vi "Main.vi"(11 "Module Admin":refnum<class "Delacor_lib_QMH_Cloneable Module Admin.lvclass">) -> ()   [LabVIEW 2020, in "reporting-device.lvlib"]
doc: "This template is based off of the Queued Message Handler design pattern and the Queued Message Handler project template that ships with LabVIEW.\n\nThe main difference is that the queue is private to this module and communication between modules is performed via Broadcast and Request events.\n\nRequest events are wrapped in public API methods and are handled in the Event Handling Loop (EHL) of this VI. Any module can register for Broadcast events sent by this module. The EHL generates messages based on user interface actions.\n\nThe Message Handling Loop (MHL) processes messages generated by the EHL, or by other messages. The messages are string values, so new messages can be added easily to the Message Cases case structure in the MHL. Each message cluster can also provide an optional value for Message Data, which is a variant that can be converted to whatever message-specific data is required.\n_____\nBased on DQMH Project Template 7.0.1.1316."
uses:
  reporting-device.lvlib
  <vilib>/Delacor/Delacor QMH/Libraries/Message Queue_class/Delacor_lib_QMH_Message Queue.lvclass
  <vilib>/Utility/miscctls.llb/LVPointTypeDef.ctl
  <vilib>/Delacor/Delacor QMH/Libraries/Message Queue_class/Delacor_lib_QMH_Enqueue Message (Single).vi
  Stop Argument--cluster.ctl
  <vilib>/Delacor/Delacor QMH/Libraries/Cloneable Module Admin_class/Delacor_lib_QMH_Cloneable Module Admin.lvclass
  connect (Reply Payload)--cluster.ctl
  connect Argument--cluster.ctl
  <userlib>/Zaphiro/GTools/Redis/Sources/Redis/Redis.lvclass
  <vilib>/Wovalab/Utilities/Helper Loop Periodic Timing/Helper Loop Periodic Timing.lvclass
  start-publishing (Reply Payload)--cluster.ctl
  start-publishing Argument--cluster.ctl
  <userlib>/Zaphiro/GTools/Time/time__ZGTools.lvlib
  <userlib>/Zaphiro/GTools/Time/public/convert lv time to unix-scalar__ZGTools.vi
  set-reporting-device (Reply Payload)--cluster.ctl
  set-reporting-device Argument--cluster.ctl
  <userlib>/Zaphiro/GTools/Time/public/convert unix time to lv-scalar__ZGTools.vi
panel:
  out "ttl":i32 format="%d s"
  out "values":dbl[](array[numeric])
  out "timestamp":timestamp format="%^<%x %.3X>T utc"
  out "latest-ts":u64
  out "info":T1
  out "status":string
  out "connected":bool
  out "error out":errorcluster
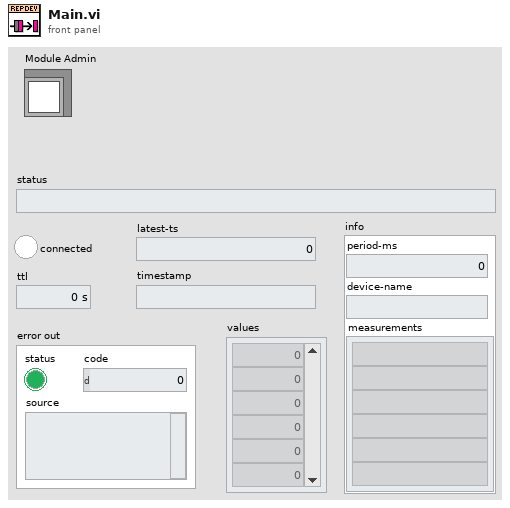
[diagram p1: front panel]
types:
  T1 = cluster{"period-ms":i32, "device-name":string, "measurements":string[]}
  T2 = typedef "reporting-device.lvlib/Request Events--cluster.ctl" = cluster{"Stop Module":refnum<user-event>, "Show Panel":refnum<user-event>, "Hide Panel":refnum<user-event>, "Show Diagram":refnum<user-event>, "Get Module Execution Status":refnum<user-event>, "connect":refnum<user-event>, "start-publishing":refnum<user-event>, "set-reporting-device":refnum<user-event>}
  T3 = typedef "reporting-device.lvlib/Module Data--cluster.ctl" = cluster{"clone-id":i32, "status":string, "dvr":cluster{"redis":refnum<data-value>}}
  T4 = enum32{"invalid lock state", "Not Locked", "Locked (No Password)", "Password-protected"}
  T5 = typedef "reporting-device.lvlib/Stop Argument--cluster.ctl" = cluster{"Module ID":i32, "Origin":string, "Exit via Stop Module Req?":bool, "Wait for Module to stop?":bool}
  T6 = typedef "reporting-device.lvlib/connect Argument--cluster.ctl" = cluster{"Module ID":i32, "flush":bool, "connection":cluster{"ip":string, "port":u16, "timeout":i32}, "Wait Notifier":refnum<notifier>, "wait for reply":bool}
  T7 = typedef "reporting-device.lvlib/start-publishing Argument--cluster.ctl" = cluster{"Module ID":i32, "Wait Notifier":refnum<notifier>, "wait for reply":bool}
  T8 = typedef "reporting-device.lvlib/set-reporting-device Argument--cluster.ctl" = cluster{"Module ID":i32, "measurement-list":string[], "period-ms":i32, "device-name":string, "ttl":i32, "Wait Notifier":refnum<notifier>, "wait for reply":bool}
  T9 = typedef "LVPointTypeDef.ctl" = cluster{"Horizontal":i16, "Vertical":i16}
  T10 = enum32{"Invalid", "Standard", "Closed", "Hidden", "Minimized", "Maximized"}
  T11 = typedef "reporting-device.lvlib/connect (Reply Payload)--cluster.ctl" = cluster{"Module ID":i32, "status":cluster{"reply-to-ping":bool, "pong":bool}, "error":errorcluster}
  T12 = typedef "reporting-device.lvlib/start-publishing (Reply Payload)--cluster.ctl" = cluster{"Module ID":i32, "ack":bool, "ts":u64, "error":errorcluster}
  T13 = typedef "reporting-device.lvlib/set-reporting-device (Reply Payload)--cluster.ctl" = cluster{"Module ID":i32, "ack":bool, "error":errorcluster}
  T14 = cluster{"output cluster":refnum<class "Redis.lvclass">}
  T15 = cluster{"period-ms":i32, "device-name":string, "measurement-list":string[]}
  T16 = cluster{u64, "device-name":string, "measurement-list":string[], "ttl":i32}
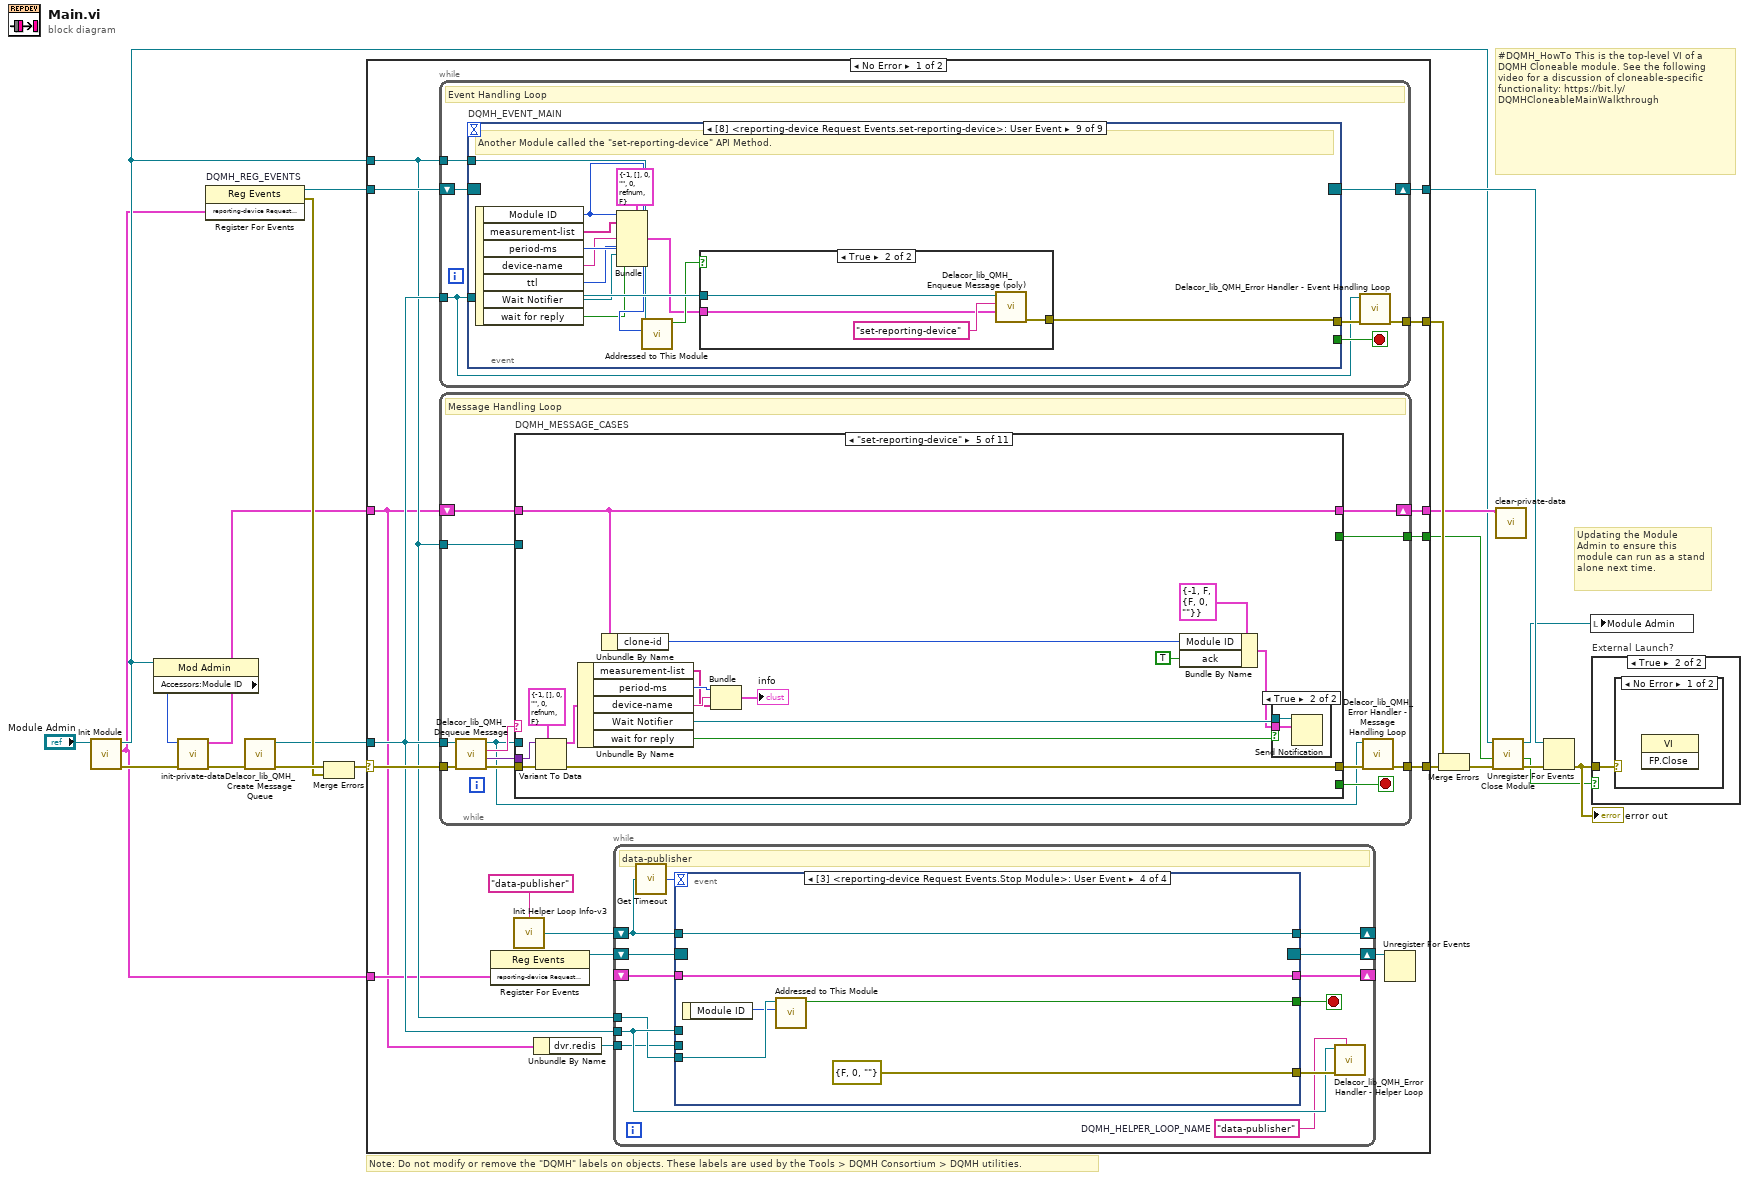
[diagram p0: block diagram]
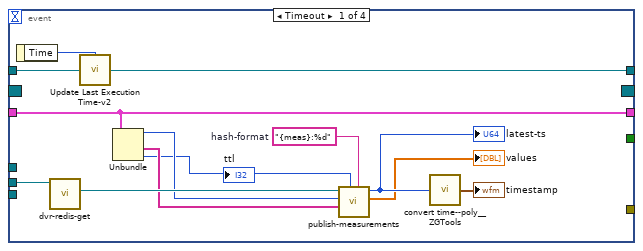
[diagram p2: hidden frame]
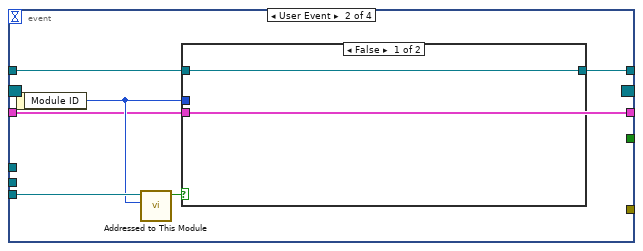
[diagram p3: hidden frame]
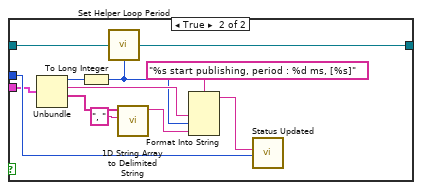
[diagram p4: hidden frame]
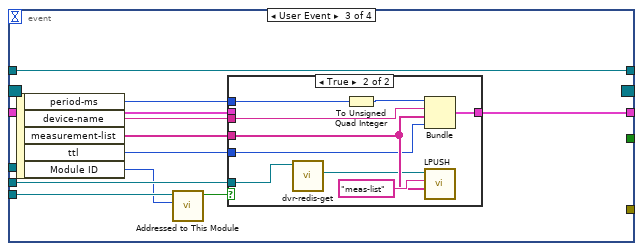
[diagram p5: hidden frame]
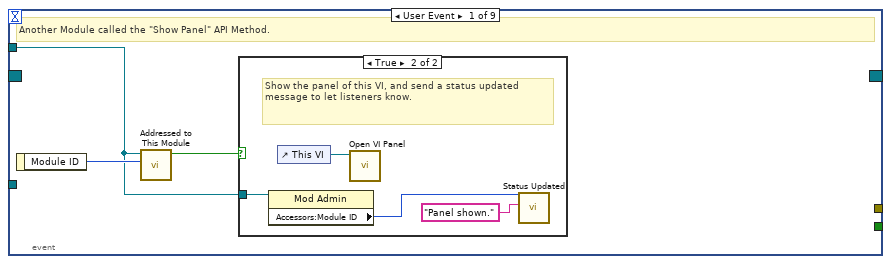
[diagram p7: hidden frame]
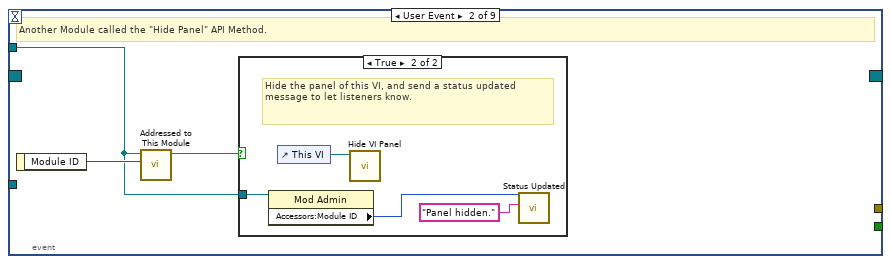
[diagram p9: hidden frame]
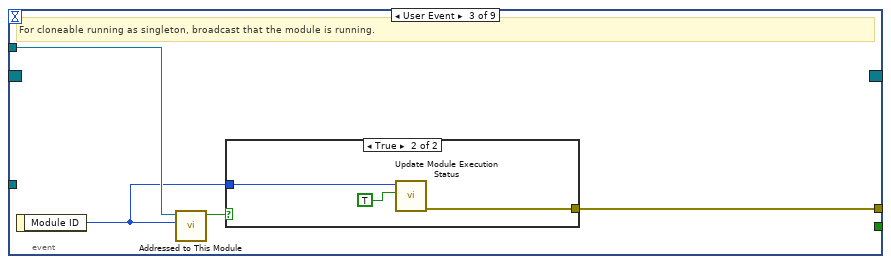
[diagram p11: hidden frame]
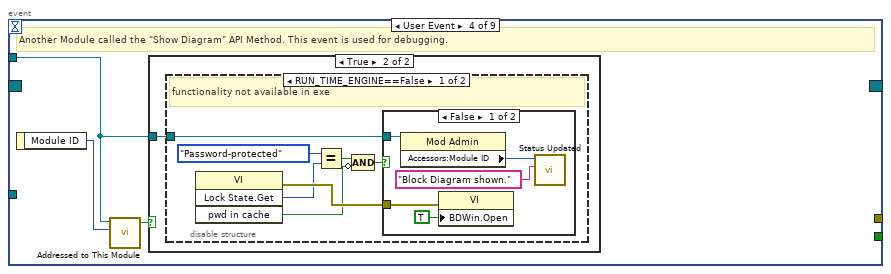
[diagram p13: hidden frame]
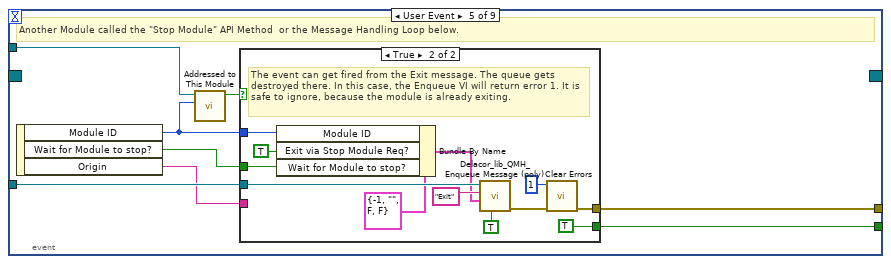
[diagram p17: hidden frame]
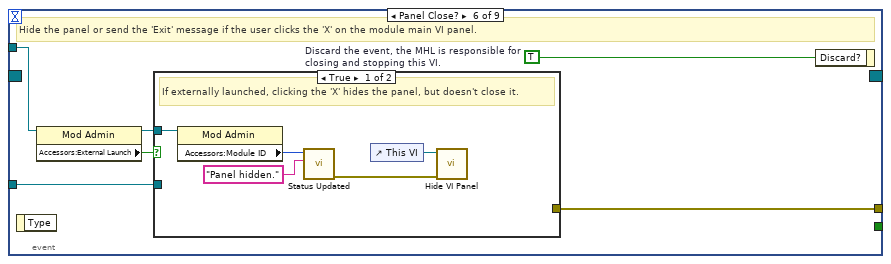
[diagram p19: hidden frame]
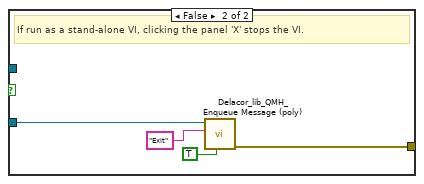
[diagram p20: hidden frame]
diagram:
  # "#DQMH_HowTo This is the top-level VI of a DQMH Cloneable module. See the following video for a discussion of cloneable-specific functionality: https://bit.ly/DQMHCloneableMainWalkthrough"
  # "Note: Do not modify or remove the \"DQMH\" labels on objects. These labels are used by the Tools > DQMH Consortium > DQMH utilities."
  # "Updating the Module Admin to ensure this module can run as a stand alone next time."
  n1 = call "Init Module.vi"("Cloneable Module Admin in"="Module Admin") -> ("error out"=w6:errorcluster, "reporting-device Request Events"=w1:T2, "Cloneable Module Admin out"=w3:refnum<class "Delacor_lib_QMH_Cloneable Module Admin.lvclass">)  [unwired: 8 in]
  n2 = property class="Mod Admin"(reference=w3) -> ("Accessors:Module ID"=w2:i32)  [unwired: 1 in, 2 out]
  n3 = call "init-private-data.vi"("error in (no error)"=w6, "clone-id"=w2) -> ("error out"=w5:errorcluster, "module-data"=w7:T3)  [unwired: 8 in]
  n4 = register-events "DQMH_REG_EVENTS"(w1) -> (reference out=w13:refnum<event-registration>, error out=w15:errorcluster)  [unwired: 2 in]
  n5 = call <vilib>:"Delacor_lib_QMH_Create Message Queue.vi"("error in"=w5) -> ("error out"=w17:errorcluster, "Message Queue"=w12:refnum<class "Delacor_lib_QMH_Message Queue.lvclass">)  [unwired: 9 in]
  n6 = Merge Errors(w17, w15) -> (w16:errorcluster)
  n7 = case shown="No Error" w16 {
    selector: w16 -> [w36 w412]
    tunnel: [w38 w411] -> w20
    tunnel: [w35 w410] -> w14
    tunnel: w13 -> [w34 w410]
    tunnel: w12 -> [w33 w403]
    tunnel: [w37 _] -> w21
    tunnel: w3 -> [w32 w406]
    tunnel: [w31 _] -> w9
    tunnel: w7 -> [w24 w402]
    tunnel: [w30 w402] -> w4
    tunnel: w1 -> [w29 _]
    frame No Error {
      n8 = while {
        tunnel: w33 -> [w111]
        shift-right: [w114] -> w35
        shift-left: w34 -> [w115]
        tunnel: [w116] -> w37
        tunnel: w32 -> [w112]
        stop <- w113 stop-if-true
        # "Event Handling Loop"
        n9 = event "DQMH_EVENT_MAIN" shown="[8] <reporting-device Request Events.set-reporting-device>: User Event" {
          selector: w115 -> [_ _ _ _ _ _ _ _ _]
          dyn-events: [_ _ _ _ _ _ _ _ _] -> w114
          timeout: _ -> [_ _ _ _ _ _ _ _ _]
          tunnel: [_ _ _ _ w158 _ _ _ _] -> w113
          tunnel: w111 -> [_ _ _ _ w161 w177 w200 w213 w230]
          tunnel: [_ _ w135 _ w162 w180 w190 w207 w221] -> w117
          tunnel: w112 -> [w118 w125 w133 w139 w160 w178 w198 w211 w228]
          event User Event {
            # "Another Module called the \"Show Panel\" API Method."
            n10 = event-data() -> ("Module ID"=w119:i32)  [unwired: 1 in]
            n11 = call "Addressed to This Module.vi"("Module ID from Argument"=w119, "Module Admin"=w118) -> ("Addressed to this instance?"=w120:bool)  [unwired: 8 in, 1 out]
            n12 = case shown="True" w120 {
              tunnel: w118 -> [_ w122]
              frame False {
              }
              frame True {
                # "Show the panel of this VI, and send a status updated message to let listeners know."
                n13 = property on="Property Node" class="Mod Admin"(reference=w122) -> ("Accessors:Module ID"=w121:i32)  [unwired: 1 in, 2 out]
                n14 = control-ref of="This VI"() -> (w124:refnum<vi>)
                n15 = call "Open VI Panel.vi"("VI"=w124) -> ()  [unwired: 10 in, 1 out]
                n16 = call "Status Updated.vi"("Status"="Panel shown." ("format string"), "Module ID"=w121) -> ()  [unwired: 9 in, 1 out]
              }
            }
          }
          event User Event {
            # "Another Module called the \"Hide Panel\" API Method."
            n17 = event-data() -> ("Module ID"=w126:i32)  [unwired: 1 in]
            n18 = call "Addressed to This Module.vi"("Module ID from Argument"=w126, "Module Admin"=w125) -> ("Addressed to this instance?"=w127:bool)  [unwired: 8 in, 1 out]
            n19 = case shown="True" w127 {
              tunnel: w125 -> [_ w129]
              frame False {
              }
              frame True {
                # "Hide the panel of this VI, and send a status updated message to let listeners know."
                n20 = property on="Property Node" class="Mod Admin"(reference=w129) -> ("Accessors:Module ID"=w128:i32)  [unwired: 1 in, 2 out]
                n21 = control-ref of="This VI"() -> (w131:refnum<vi>)
                n22 = call "Hide VI Panel.vi"("VI"=w131) -> ()  [unwired: 10 in, 1 out]
                n23 = call "Status Updated.vi"("Status"="Panel hidden." ("format string"), "Module ID"=w128) -> ()  [unwired: 9 in, 1 out]
              }
            }
          }
          event User Event {
            # "For cloneable running as singleton, broadcast that the module is running."
            n24 = event-data() -> ("Module ID"=w132:i32)  [unwired: 1 in]
            n25 = call "Addressed to This Module.vi"("Module ID from Argument"=w132, "Module Admin"=w133) -> ("Addressed to this instance?"=w134:bool)  [unwired: 8 in, 1 out]
            n26 = case shown="True" w134 {
              tunnel: [_ w138] -> w135
              tunnel: w132 -> [_ w137]
              frame False {
              }
              frame True {
                n27 = call "Update Module Execution Status.vi"("Running?"=TRUE, "Module ID"=w137) -> ("error out"=w138:errorcluster)  [unwired: 9 in]
              }
            }
          }
          event User Event {
            # "Another Module called the \"Show Diagram\" API Method. This event is used for debugging."
            n28 = event-data() -> ("Module ID"=w140:i32)  [unwired: 1 in]
            n29 = call "Addressed to This Module.vi"("Module ID from Argument"=w140, "Module Admin"=w139) -> ("Addressed to this instance?"=w141:bool)  [unwired: 8 in, 1 out]
            n30 = case shown="True" w141 {
              tunnel: w139 -> [_ w142]
              frame False {
              }
              frame True {
                n31 = disable-structure shown="RUN_TIME_ENGINE==False" {
                  disable-tunnel: w142 -> [w143 _]
                  frame condition #0 (active) {
                    # "functionality not available in exe"
                    n32 = invoke on="Invoke Node" class="VI" method="Lock State.Get"() -> (error out=w149:errorcluster, "Get Lock State"=w148:T4, "pwd in cache"=w145:bool)  [unwired: 4 in, 1 out]
                    n33 = Equal?(x=T4."Password-protected", y=w148) -> (x = y?=w146:bool)
                    n34 = Compound Arithmetic op=AND(w146, invert w145) -> (w144:bool)
                    n35 = case shown="False" w144 {
                      tunnel: w149 -> [w154 _]
                      tunnel: w143 -> [w151 _]
                      frame False {
                        n36 = property on="Property Node" class="Mod Admin"(reference=w151) -> ("Accessors:Module ID"=w150:i32)  [unwired: 1 in, 2 out]
                        n37 = property on="Property Node" class="VI"(error in=w154, "BDWin.Open"=TRUE ("Block Diagram Window:Open")) -> ()  [unwired: 1 in, 2 out]
                        n38 = call "Status Updated.vi"("Status"="Block Diagram shown." ("format string"), "Module ID"=w150) -> ()  [unwired: 9 in, 1 out]
                      }
                      frame True {
                        # "Password-protected VI, and the password is not in the cache. Do not show the diagram."
                      }
                    }
                  }
                  frame condition #1 {
                  }
                }
              }
            }
          }
          event User Event {
            # "Another Module called the \"Stop Module\" API Method  or the Message Handling Loop below."
            n39 = event-data() -> ("Module ID"=w156:i32, "Wait for Module to stop?"=w157:bool, "Origin"=w155:string)  [unwired: 1 in]
            n40 = call "Addressed to This Module.vi"("Module ID from Argument"=w156, "Module Admin"=w160) -> ("Addressed to this instance?"=w159:bool)  [unwired: 8 in, 1 out]
            n41 = case shown="True" w159 {
              tunnel: [_ w173] -> w162
              tunnel: w161 -> [_ w169]
              tunnel: [_ TRUE] -> w158
              tunnel: w157 -> [_ w164]
              tunnel: w156 -> [_ w166]
              tunnel: w155 -> [_ _]
              frame False {
              }
              frame True {
                # "The event can get fired from the Exit message. The queue gets destroyed there. In this case, the Enqueue VI will return error 1. It is safe to ignore, because the module is already exiting."
                n42 = Bundle By Name(cluster=T5 {"Module ID"=-1, "Origin"="", "Exit via Stop Module Req?"=FALSE, "Wait for Module to stop?"=FALSE} ("Stop Argument"), "Module ID"=w166, "Exit via Stop Module Req?"=TRUE, "Wait for Module to stop?"=w164) -> (w163:T5)
                n43 = call-poly <vilib>:"Delacor_lib_QMH_Enqueue Message (poly).vi"("Priority Message? (F)"=TRUE, "Message Data"=w163, "Message"="Exit", "Message Queue in"=w169) -> ("error out"=w174:errorcluster)  [unwired: 6 in, 1 out]
                n44 = call <vilib>:"Clear Errors.vi"("error in (no error)"=w174, "specific error code to clear (0: all)"=1) -> ("error out"=w173:errorcluster)  [unwired: 4 in, 1 out]
              }
            }
          }
          event Panel Close? {
            w179 = TRUE  # Discard the event, the MHL is responsible for closing and stopping this VI.
            # "Hide the panel or send the 'Exit' message if the user clicks the 'X' on the module main VI panel."
            n45 = event-data() -> ()  [unwired: 1 in, 1 out]
            n46 = property on="Property Node" class="Mod Admin"(reference=w178) -> (reference out=w175:refnum<class "Delacor_lib_QMH_Cloneable Module Admin.lvclass">, "Accessors:External Launch"=w176:bool)  [unwired: 1 in, 1 out]
            n47 = case shown="True" w176 {
              tunnel: w177 -> [_ w188]
              tunnel: [_ w189] -> w180
              tunnel: w175 -> [w183 _]
              frame True {
                # "If externally launched, clicking the 'X' hides the panel, but doesn't close it."
                n48 = property on="Property Node" class="Mod Admin"(reference=w183) -> ("Accessors:Module ID"=w182:i32)  [unwired: 1 in, 2 out]
                n49 = call "Status Updated.vi"("Status"="Panel hidden." ("format string"), "Module ID"=w182) -> ("error out"=w181:errorcluster)  [unwired: 9 in]
                n50 = control-ref of="This VI"() -> (w185:refnum<vi>)
                n51 = call "Hide VI Panel.vi"("error in"=w181, "VI"=w185) -> ()  [unwired: 9 in, 1 out]
              }
              frame False {
                # "If run as a stand-alone VI, clicking the panel 'X' stops the VI."
                n52 = call-poly <vilib>:"Delacor_lib_QMH_Enqueue Message (poly).vi"("Priority Message? (F)"=TRUE, "Message"="Exit", "Message Queue in"=w188) -> ("error out"=w189:errorcluster)  [unwired: 7 in, 1 out]
              }
            }
            n53 = event-data ("Event Filter Node")("Discard?"=w179) -> ()  [unwired: 1 in, 1 out]
          }
          event User Event {
            # "Another Module called the \"connect\" API Method."
            n54 = event-data() -> ("Module ID"=w195:i32, "flush"=w194:bool, "connection"=w193:cluster{"ip":string, "port":u16, "timeout":i32}, "Wait Notifier"=w192:refnum<notifier>, "wait for reply"=w191:bool)  [unwired: 1 in]
            n55 = Bundle(cluster=T6 {"Module ID"=-1, "flush"=FALSE, "connection"={"ip"="localhost", "port"=6379, "timeout"=1000}, "Wait Notifier"=refnum, "wait for reply"=FALSE} ("connect Argument"), "Module ID"=w195, "flush"=w194, "connection"=w193, "Wait Notifier"=w192, "wait for reply"=w191) -> (w196:T6)
            n56 = call "Addressed to This Module.vi"("Module ID from Argument"=w195, "Module Admin"=w198) -> ("Addressed to this instance?"=w199:bool)  [unwired: 8 in, 1 out]
            n57 = case shown="True" w199 {
              tunnel: w200 -> [_ w204]
              tunnel: w196 -> [_ w202]
              tunnel: [_ w201] -> w190
              frame False {
              }
              frame True {
                n58 = call-poly <vilib>:"Delacor_lib_QMH_Enqueue Message (poly).vi"("Message Data"=w202, "Message"="connect", "Message Queue in"=w204) -> ("error out"=w201:errorcluster)  [unwired: 7 in, 1 out]
              }
            }
          }
          event User Event {
            # "Another Module called the \"start-publishing\" API Method."
            n59 = event-data() -> ("Module ID"=w208:i32, "Wait Notifier"=w205:refnum<notifier>, "wait for reply"=w206:bool)  [unwired: 1 in]
            n60 = Bundle(cluster=T7 {"Module ID"=-1, "Wait Notifier"=refnum, "wait for reply"=FALSE} ("start-publishing Argument"), "Module ID"=w208, "Wait Notifier"=w205, "wait for reply"=w206) -> (w209:T7)
            n61 = call "Addressed to This Module.vi"("Module ID from Argument"=w208, "Module Admin"=w211) -> ("Addressed to this instance?"=w212:bool)  [unwired: 8 in, 1 out]
            n62 = case shown="True" w212 {
              tunnel: w213 -> [_ w217]
              tunnel: w209 -> [_ w215]
              tunnel: [_ w214] -> w207
              frame False {
              }
              frame True {
                n63 = call-poly <vilib>:"Delacor_lib_QMH_Enqueue Message (poly).vi"("Message Data"=w215, "Message"="start-publishing", "Message Queue in"=w217) -> ("error out"=w214:errorcluster)  [unwired: 7 in, 1 out]
              }
            }
          }
          event User Event {
            # "Another Module called the \"set-reporting-device\" API Method."
            n64 = event-data() -> ("Module ID"=w225:i32, "measurement-list"=w224:string[], "period-ms"=w223:i32, "device-name"=w222:string, "ttl"=w220:i32, "Wait Notifier"=w219:refnum<notifier>, "wait for reply"=w218:bool)  [unwired: 1 in]
            n65 = Bundle(cluster=T8 {"Module ID"=-1, "measurement-list"=[], "period-ms"=0, "device-name"="", "ttl"=0, "Wait Notifier"=refnum, "wait for reply"=FALSE} ("set-reporting-device Argument"), "Module ID"=w225, "measurement-list"=w224, "period-ms"=w223, "device-name"=w222, "ttl"=w220, "Wait Notifier"=w219, "wait for reply"=w218) -> (w226:T8)
            n66 = call "Addressed to This Module.vi"("Module ID from Argument"=w225, "Module Admin"=w228) -> ("Addressed to this instance?"=w229:bool)  [unwired: 8 in, 1 out]
            n67 = case shown="True" w229 {
              tunnel: w230 -> [_ w234]
              tunnel: w226 -> [_ w232]
              tunnel: [_ w231] -> w221
              frame False {
              }
              frame True {
                n68 = call-poly <vilib>:"Delacor_lib_QMH_Enqueue Message (poly).vi"("Message Data"=w232, "Message"="set-reporting-device", "Message Queue in"=w234) -> ("error out"=w231:errorcluster)  [unwired: 7 in, 1 out]
              }
            }
          }
        }
        n69 = call-dynamic "Delacor_lib_QMH_Error Handler - Event Handling Loop.vi"("error in"=w117, "Message Queue in"=w111) -> ("dup error in"=w116:errorcluster)  [unwired: 8 in, 1 out]
      }
      n70 = while {
        tunnel: w33 -> [w235]
        shift-right: [w242] -> w30
        shift-left: w24 -> [w243]
        tunnel: w36 -> [w246]
        tunnel: [w244] -> w38
        tunnel: w32 -> [w237]
        tunnel: [w236] -> w31
        stop <- w241 stop-if-true
        # "Message Handling Loop"
        n71 = call-dynamic "Delacor_lib_QMH_Dequeue Message.vi"("error in"=w246, "Message Queue in"=w235) -> ("error out"=w245:errorcluster, "Message Data"=w239:variant, "Message"=w240:string, "Message Queue out"=w238:refnum<class "Delacor_lib_QMH_Message Queue.lvclass">)  [unwired: 6 in]
        n72 = case "DQMH_MESSAGE_CASES" shown="\"set-reporting-device\"" w240 {
          selector: w240 -> [_ _ _ _ _ _ _ _ _ _ w394]
          tunnel: w238 -> [_ _ _ _ _ _ _ w345 _ w382 _]
          tunnel: w245 -> [w266 w270 w295 w316 w334 w339 w341 w353 w369 w388 w400]
          tunnel: [w264 w270 w282 w308 w321 w338 w341 w349 w368 w383 w401] -> w247
          tunnel: w243 -> [w249 w269 w281 w303 w320 w337 w340 w343 w361 w373 w392]
          tunnel: [w257 w269 w281 w303 w320 w337 w340 w343 w361 w373 w392] -> w242
          tunnel: [_ _ _ _ _ _ _ _ _ w381 _] -> w241
          tunnel: w239 -> [_ _ w294 w315 w333 _ _ w348 _ w379 _]
          tunnel: w237 -> [w253 _ _ _ _ _ _ w347 _ w374 _]
          tunnel: [_ _ _ _ _ _ _ _ _ w377 _] -> w236
          frame "Initialize" {
            # "#CodeNeeded - Initialize the appearance of the front panel."
            # "#CodeNeeded - Initialize your state data here."
            # "Initialize - Any operation that needs to be done before the module can receive messages. Synchronize Caller Events.vi will inform Start Module.vi that the module has launched and is ready to receive messages. Module Did Init.vi will broadcast that the module initialized."
            n73 = call "Synchronize Caller Events.vi"("error in"=w266, "Module Admin"=w253) -> ("error out"=w265:errorcluster, "Module Admin out"=w252:refnum<class "Delacor_lib_QMH_Cloneable Module Admin.lvclass">)  [unwired: 8 in]
            n74 = property on="Property Node" class="Mod Admin"(reference=w252) -> ("Accessors:External Launch"=w254:bool)  [unwired: 1 in, 2 out]
            n75 = Unbundle By Name(w249) -> ("clone-id"=w248:i32)
            n76 = call "Module Name--constant.vi"("Module ID"=w248) -> ("Module Name"=w261:string)  [unwired: 10 in]
            n77 = property on="Property Node" class="VI"("Front Panel.Title"=w261) -> (reference out=w263:refnum<vi>, error out=w268:errorcluster)  [unwired: 2 in]
            n78 = Select(t=T10."Hidden" ("State"), s=w254, f=T10."Standard" ("State")) -> (s? t:f=w258:T10)
            n79 = invoke on="Invoke Node" class="VI" method="FP.Open"(reference=w263, error in=w268, "State"=w258) -> (reference out=w262:refnum<vi>, error out=w267:errorcluster)  [unwired: 2 in, 3 out]
            n80 = call "Module Name--constant.vi"("Module ID"=w248) -> ("Module Name"=w255:string)  [unwired: 10 in]
            n81 = Bundle By Name(cluster=w249, "status"="Initial Message" ("Initial Message")) -> (w257:T3)
            n82 = invoke on="Invoke Node" class="VI" method="FP.Center"(reference=w262, error in=w267) -> ()  [unwired: 1 in, 3 out]
            n83 = property on="Pane" class="Pane"("Origin"=T9 {"Horizontal"=0, "Vertical"=0}) -> ()  [unwired: 2 in, 2 out]
            n84 = call "Module Did Init.vi"("error in"=w265, "Initialized?"=TRUE, "Origin"=w255, "Module ID"=w248) -> ("error out"=w264:errorcluster)  [unwired: 7 in]
          }
          frame "---Module Specific---" {
            # "Separator -- The following cases handle messages specific to this Module."
          }
          frame "connect" {
            w283 = TRUE  # #oneday
            # "connect to a redis instance"
            n85 = Variant To Data(error in=w295, type=T6 {"Module ID"=-1, "flush"=FALSE, "connection"={"ip"="localhost", "port"=6379, "timeout"=1000}, "Wait Notifier"=refnum, "wait for reply"=FALSE} ("connect Argument"), Variant=w294) -> (data=w292:T6, error out=w282:errorcluster)
            n86 = Unbundle By Name(w292) -> ("flush"=w287:bool, "connection"=w286:cluster{"ip":string, "port":u16, "timeout":i32}, "Wait Notifier"=w291:refnum<notifier>, "wait for reply"=w290:bool)
            n87 = Unbundle By Name(w286) -> ("ip"=w277:string, "port"=w276:u16, "timeout"=w285:i32)
            n88 = Unbundle By Name(w281) -> ("clone-id"=w278:i32, "dvr.redis"=w280:refnum<data-value>)
            n89 = call <userlib>:"Open_Redis.vi"("Flush Stack befor each cmd"=w287, "Tcp timeout ms"=w285, "Port"=w276, "Host"=w277) -> ("error out"=w284:errorcluster, "connection-ok"=w275:bool, "output cluster"=w279:refnum<class "Redis.lvclass">)  [unwired: 5 in]
            "connected" <- w275
            n90 = case shown="True" w275 {
              tunnel: w280 -> [_ w296]
              tunnel: w279 -> [_ w297]
              frame False {
              }
              frame True {
                n91 = in-place {
                  in-place-border: w297 -> [w299]
                  n92 = in-place-dvr #1(w296) -> ()  [unwired: 2 out]
                  n93 = Bundle("output cluster"=w299) -> (w298:T14)  [unwired: 1 in]
                  n94 = in-place-dvr #1(w298) -> ()  [unwired: 2 out]
                }
              }
            }
            n95 = Select(t="connected to %s:%d" ("format string"), s=w275, f="failed to connect to %s:%d" ("format string")) -> (s? t:f=w272:string)
            n96 = Format Into String(format string=w272, w277, w276) -> (resulting string=w271:string)  [unwired: 2 in, 1 out]
            "status" <- w271
            n97 = Bundle By Name(cluster=T11 {"Module ID"=-1, "status"={"reply-to-ping"=FALSE, "pong"=FALSE}, "error"={"status"=FALSE, "code"=0, "source"=""}} ("connect (Reply Payload)"), "Module ID"=w278, "status.reply-to-ping"=w283, "status.pong"=w275, "error"=w284) -> (w289:T11)
            n98 = call "Status Updated.vi"("Status"=w271, "Module ID"=w278) -> ()  [unwired: 9 in, 1 out]
            n99 = case "DQMH_FIRE_NOTIFIER" shown="True" w290 {
              tunnel: w291 -> [_ w301]
              tunnel: w289 -> [_ w300]
              frame False {
              }
              frame True {
                n100 = Send Notification(notification=w300, notifier=w301) -> ()  [unwired: 1 in, 2 out]
              }
            }
          }
          frame "start-publishing" {
            # "start data publishing at given period the given meausrement list"
            n101 = Variant To Data(error in=w316, type=T7 {"Module ID"=-1, "Wait Notifier"=refnum, "wait for reply"=FALSE} ("start-publishing Argument"), Variant=w315) -> (data=w313:T7, error out=w308:errorcluster)
            n102 = Unbundle By Name(w313) -> ("Wait Notifier"=w312:refnum<notifier>, "wait for reply"=w311:bool)
            n103 = Unbundle By Name(w303) -> ("clone-id"=w302:i32)
            n104 = Get Date/Time In Seconds() -> (seconds since 1Jan1904=w305:timestamp)
            n105 = call-poly <userlib>:"convert time--poly__ZGTools.vi"("labview-timestamp"=w305) -> ("unix-time"=w304:u64)  [unwired: 8 in]
            n106 = Bundle By Name(cluster=T12 {"Module ID"=-1, "ack"=FALSE, "ts"=0, "error"={"status"=FALSE, "code"=0, "source"=""}} ("start-publishing (Reply Payload)"), "Module ID"=w302, "ack"=TRUE, "ts"=w304, "error"=errorcluster {"status"=FALSE, "code"=0, "source"=""}) -> (w310:T12)
            n107 = case "DQMH_FIRE_NOTIFIER" shown="True" w311 {
              tunnel: w312 -> [_ w318]
              tunnel: w310 -> [_ w317]
              frame False {
              }
              frame True {
                n108 = Send Notification(notification=w317, notifier=w318) -> ()  [unwired: 1 in, 2 out]
              }
            }
          }
          frame "set-reporting-device" {
            n109 = Variant To Data(error in=w334, type=T8 {"Module ID"=-1, "measurement-list"=[], "period-ms"=0, "device-name"="", "ttl"=0, "Wait Notifier"=refnum, "wait for reply"=FALSE} ("set-reporting-device Argument"), Variant=w333) -> (data=w331:T8, error out=w321:errorcluster)
            n110 = Unbundle By Name(w331) -> ("measurement-list"=w323:string[], "period-ms"=w325:i32, "device-name"=w324:string, "Wait Notifier"=w330:refnum<notifier>, "wait for reply"=w329:bool)
            n111 = Unbundle By Name(w320) -> ("clone-id"=w319:i32)
            n112 = Bundle("period-ms"=w325, "device-name"=w324, "measurement-list"=w323) -> (→"info":T15)  [unwired: 1 in]
            n113 = Bundle By Name(cluster=T13 {"Module ID"=-1, "ack"=FALSE, "error"={"status"=FALSE, "code"=0, "source"=""}} ("set-reporting-device (Reply Payload)"), "Module ID"=w319, "ack"=TRUE) -> (w328:T13)
            n114 = case "DQMH_FIRE_NOTIFIER" shown="True" w329 {
              tunnel: w330 -> [_ w336]
              tunnel: w328 -> [_ w335]
              frame False {
              }
              frame True {
                n115 = Send Notification(notification=w335, notifier=w336) -> ()  [unwired: 1 in, 2 out]
              }
            }
          }
          frame "---Copy This Frame---" {
            # "Duplicate this frame when creating new messages.  Change this comment in the duplicated frame to describe this message."
            n116 = Merge Errors(w339) -> (w338:errorcluster)
          }
          frame "---Exit and Error Handling---" {
            # "Separator - the following cases handle errors and exit messages."
          }
          frame "Error" {
            # "#CodeRecommended - If the module is running in standalone mode (External Launch = FALSE), this code will pop up an error dialog and call the 'Exit' message if an error occurs. Add more fine-grained error management here."
            # "Error - Check the error message data and respond accordingly. This message is sent by the \"Error Handler\" VIs at the end of each loop in this application."
            n117 = property on="Property Node" class="Mod Admin"(reference=w347) -> ("Accessors:External Launch"=w346:bool)  [unwired: 1 in, 2 out]
            n118 = Variant To Data(error in=w353, type=errorcluster {"status"=FALSE, "code"=0, "source"=""} ("error constant"), Variant=w348) -> (data=w344:errorcluster, error out=w351:errorcluster)
            n119 = Unbundle By Name(w343) -> ("clone-id"=w342:i32)
            n120 = local write "error out"(w344) -> ()
            n121 = call "Error Reported.vi"("Error"=w344, "Module ID"=w342) -> ()  [unwired: 9 in, 1 out]
            n122 = case shown="False" w346 {
              tunnel: [w358 _] -> w350
              tunnel: w345 -> [w356 _]
              tunnel: w344 -> [w357 _]
              frame False {
                n123 = disable-structure shown="Default" {
                  disable-tunnel: w357 -> [w359 _]
                  frame condition #0 (active) {
                    # "If the module is running standalone, then pop up an error dialog and call the \"Exit\" message."
                    n124 = call <vilib>:"Simple Error Handler.vi"("error in (no error)"=w359) -> ()  [unwired: 4 in, 5 out]
                  }
                  frame condition #1 {
                    # "To prevent the Simple Error Handler VI from being loaded (e.g. when deploying to a Real-Time target), add the Conditional Disable Symbol \"DQMH_Disable_SEH\" to your project and set it to TRUE."
                  }
                }
                n125 = call-poly <vilib>:"Delacor_lib_QMH_Enqueue Message (poly).vi"("Priority Message? (F)"=TRUE, "Message"="Exit", "Message Queue in"=w356) -> ("error out"=w358:errorcluster)  [unwired: 7 in, 1 out]
              }
              frame True {
                # "If the module was launched externally, calling the Error Reported broadcast VI is the only action performed by the \"Error\" message. The module's caller can then process the error appropriately."
              }
            }
            n126 = Merge Errors(w351, w350) -> (w349:errorcluster)
          }
          frame "Simulate MHL Error" {
            # "#DQMH_HowTo The 'Simulate MHL Error' button  illustrates how the MHL handles errors. This event is instructional in nature and can be removed."
            # "Simulate an error occurring at the MHL"
            n127 = Unbundle By Name(w361) -> ("clone-id"=w360:i32)
            n128 = call "Module Name--constant.vi"("Module ID"=w360) -> ("Module Name"=w363:string)  [unwired: 10 in]
            n129 = Format Into String(format string="Simulated error originating at Message Handling Loop in %s", w363) -> (resulting string=w364:string)  [unwired: 2 in, 1 out]
            n130 = call <vilib>:"Error Cluster From Error Code.vi"("show call chain? (False)"=TRUE, "error message (\"\")"=w364, "error code (0)"=5001) -> ("error out"=w367:errorcluster)  [unwired: 6 in]
            n131 = Merge Errors(w369, w367) -> (w368:errorcluster)
          }
          frame "Exit" {
            w380 = 91  # 91: not all Exit messages will have an argument
            w381 = TRUE  # Stop the VI
            # "Release the message queue reference"
            # "#CodeNeeded - Add any required cleanup code here."
            # "Exit - Exit the application."
            n132 = Variant To Data(error in=w388, type=T5 {"Module ID"=-1, "Origin"="", "Exit via Stop Module Req?"=FALSE, "Wait for Module to stop?"=FALSE} ("Stop Argument"), Variant=w379) -> (data=w376:T5, error out=w384:errorcluster)
            n133 = call <vilib>:"Clear Errors.vi"("error in (no error)"=w384, "specific error code to clear (0: all)"=w380) -> ("error out"=w387:errorcluster)  [unwired: 4 in, 1 out]
            n134 = Unbundle By Name(w373) -> ("clone-id"=w372:i32, "dvr.redis"=w371:refnum<data-value>)
            n135 = control-ref of="This VI"() -> (w375:refnum<vi>)
            n136 = call-dynamic "Delacor_lib_QMH_Release Message Queue.vi"("error in"=w387, "Message Queue"=w382) -> ("error out"=w386:errorcluster)  [unwired: 9 in]
            n137 = call "Handle Exit.vi"("Stop Argument"=w376, "Module Admin in"=w374, "VI reference"=w375) -> ("error out"=w385:errorcluster, "Wait for Stop?"=w377:bool)  [unwired: 7 in]
            n138 = in-place {
              in-place-border: [w389] -> w370
              n139 = in-place-dvr #2(w371) -> (w390:T14)  [unwired: 1 out]
              n140 = Unbundle(w390) -> ("output cluster"=w389:refnum<class "Redis.lvclass">)
              n141 = in-place-dvr #2() -> ()  [unwired: 1 in, 2 out]
            }
            n142 = Merge Errors(w386, w385) -> (w383:errorcluster)
            n143 = call "Error Reported.vi"("Error"=w383, "Module ID"=w372) -> ()  [unwired: 9 in, 1 out]
            n144 = call <userlib>:"Close_Redis.vi"("Redis.lvclass in"=w370) -> ()  [unwired: 9 in, 2 out]
          }
          frame Default {
            # "'Default' case only runs if there is a message that isn't defined in any of the other cases.  Output a programming error."
            n145 = Unbundle By Name(w392) -> ("clone-id"=w391:i32)
            n146 = call "Module Name--constant.vi"("Module ID"=w391) -> ("Module Name"=w393:string)  [unwired: 10 in]
            n147 = Format Into String(format string="The invalid message string \"%s\" was received in the Message Handling Loop for module \"%s\".", w394, w393) -> (resulting string=w396:string)  [unwired: 2 in, 1 out]
            n148 = call <vilib>:"Error Cluster From Error Code.vi"("show call chain? (False)"=TRUE, "error message (\"\")"=w396, "error code (0)"=1) -> ("error out"=w399:errorcluster)  [unwired: 6 in]
            n149 = Merge Errors(w400, w399) -> (w401:errorcluster)
          }
        }
        n150 = call-dynamic "Delacor_lib_QMH_Error Handler - Message Handling Loop.vi"("error in"=w247, "Message Queue in"=w238) -> ("dup error in"=w244:errorcluster)  [unwired: 8 in, 1 out]
      }
      n151 = register-events ("DQMH_HELPER_REGFOREVENTS")(w29) -> (reference out=w27:refnum<event-registration>)  [unwired: 2 in, 1 out]
      n152 = call <vilib>:"Init Helper Loop Info-v3.vi"("Loop Name (\"\": Caller VI)"="data-publisher" ("Loop Name (\"\": Caller VI)")) -> ("Helper Loop Periodic Timing"=w25:refnum<class "Helper Loop Periodic Timing.lvclass">)  [unwired: 1 in]
      n153 = Unbundle By Name(w24) -> ("dvr.redis"=w23:refnum<data-value>)
      n154 = while "DQMH_HELPER_LOOP" {
        shift-right: [w51] -> _
        shift-left: w25 -> [w43]
        shift-right: [w49] -> w28
        shift-left: w27 -> [w50]
        tunnel: w33 -> [w46]
        tunnel: w32 -> [w44]
        shift-right: [w41] -> _
        shift-left: _ -> [w40]
        tunnel: w23 -> [w39]
        stop <- w48 stop-if-true
        w45 = "data-publisher"  # DQMH_HELPER_LOOP_NAME
        # "data-publisher"
        n155 = call <vilib>:"Get Timeout.vi"("Helper Loop Periodic Timing"=w43) -> ("Timeout (ms)"=w42:i32)  [unwired: 12 in, 2 out]
        n156 = event "DQMH_HELPER_EVENT_STRUCTURE" shown="[3] <reporting-device Request Events.Stop Module>: User Event" {
          selector: w50 -> [_ _ _ _]
          dyn-events: [_ _ _ _] -> w49
          timeout: w42 -> [_ _ _ _]
          tunnel: w43 -> [w63 w70 w89 w110]
          tunnel: [w64 w69 w89 w110] -> w51
          tunnel: [_ _ _ w107] -> w48
          tunnel: [_ _ _ errorcluster {"status"=FALSE, "code"=0, "source"=""} ("error constant")] -> w47
          tunnel: w46 -> [_ _ _ _]
          tunnel: w44 -> [_ w68 w94 w108]
          tunnel: [w62 w65 w91 w105] -> w41
          tunnel: w39 -> [w61 _ w86 _]
          tunnel: w40 -> [w62 w65 w90 w105]
          event Timeout {
            w58 = "{meas}:%d"  # hash-format
            n157 = event-data() -> ("Time"=w55:u32)  [unwired: 1 in]
            n158 = call "dvr-redis-get.vi"("redis-dvr"=w61) -> ("Redis out"=w60:refnum<class "Redis.lvclass">)  [unwired: 10 in]
            n159 = call <vilib>:"Update Last Execution Time-v2.vi"("Time"=w55, "Helper Loop Periodic Timing in"=w63) -> ("Helper Loop Periodic Timing out"=w64:refnum<class "Helper Loop Periodic Timing.lvclass">)  [unwired: 12 in, 1 out]
            n160 = Unbundle(w62) -> (w56:u64, "measurement-list"=w59:string[], "ttl"=w52:i32)  [unwired: 1 out]
            "ttl" <- w52
            n161 = call "publish-measurements.vi"("hash-format"=w58, "ttl"=w52, "measurement-list"=w59, "period"=w56, "Redis in"=w60) -> ("values"=→"values":dbl[], "unix-time"=w54:u64)  [unwired: 4 in, 1 out]
            "latest-ts" <- w54
            n162 = call-poly <userlib>:"convert time--poly__ZGTools.vi"("unix-time"=w54) -> ("labview-timestamp"=→"timestamp":timestamp)  [unwired: 8 in]
          }
          event User Event {
            n163 = event-data() -> ("Module ID"=w66:i32)  [unwired: 1 in]
            n164 = call "Addressed to This Module.vi"("Module ID from Argument"=w66, "Module Admin"=w68) -> ("Addressed to this instance?"=w67:bool)  [unwired: 8 in, 1 out]
            n165 = case shown="False" w67 {
              tunnel: w70 -> [w71 w83]
              tunnel: [w71 w82] -> w69
              tunnel: w65 -> [_ w76]
              tunnel: w66 -> [_ w77]
              frame False {
              }
              frame True {
                n166 = Unbundle(w76) -> (w75:u64, "device-name"=w74:string, "measurement-list"=w73:string[])  [unwired: 1 out]
                n167 = To Long Integer(number=w75) -> (32bit integer=w72:i32)
                n168 = call <vilib>:"Set Helper Loop Period.vi"("Period (ms)"=w72, "Helper Loop Periodic Timing in"=w83) -> ("Helper Loop Periodic Timing out"=w82:refnum<class "Helper Loop Periodic Timing.lvclass">)  [unwired: 13 in]
                n169 = call <vilib>:"1D String Array to Delimited String.vi"("delimiter"=", ", "string array"=w73) -> ("delimited string"=w80:string)  [unwired: 9 in]
                n170 = Format Into String(format string="%s start publishing, period : %d ms, [%s]", w74, w72, w80) -> (resulting string=w81:string)  [unwired: 2 in, 1 out]
                n171 = call "Status Updated.vi"("Status"=w81, "Module ID"=w77) -> ()  [unwired: 9 in, 1 out]
              }
            }
          }
          event User Event {
            n172 = event-data() -> ("period-ms"=w92:i32, "device-name"=w88:string, "measurement-list"=w87:string[], "ttl"=w85:i32, "Module ID"=w84:i32)  [unwired: 1 in]
            n173 = call "Addressed to This Module.vi"("Module ID from Argument"=w84, "Module Admin"=w94) -> ("Addressed to this instance?"=w93:bool)  [unwired: 8 in, 1 out]
            n174 = case shown="True" w93 {
              tunnel: w92 -> [_ w103]
              tunnel: [w95 w104] -> w91
              tunnel: w90 -> [w95 _]
              tunnel: w88 -> [_ w102]
              tunnel: w87 -> [_ w98]
              tunnel: w86 -> [_ w100]
              tunnel: w85 -> [_ w96]
              frame False {
              }
              frame True {
                n175 = call "dvr-redis-get.vi"("redis-dvr"=w100) -> ("Redis out"=w97:refnum<class "Redis.lvclass">)  [unwired: 10 in]
                n176 = To Unsigned Quad Integer(1:w103) -> (0:w101:u64)
                n177 = Bundle(w101, "device-name"=w102, "measurement-list"=w98, "ttl"=w96) -> (w104:T16)  [unwired: 1 in]
                n178 = call <userlib>:"LPUSH.vi"("Elements"=w98, "Key"="meas-list", "Redis.lvclass in"=w97) -> ()  [unwired: 6 in, 3 out]
              }
            }
          }
          event User Event {
            n179 = event-data() -> ("Module ID"=w106:i32)  [unwired: 1 in]
            n180 = call "Addressed to This Module.vi"("Module ID from Argument"=w106, "Module Admin"=w108) -> ("Addressed to this instance?"=w107:bool)  [unwired: 8 in, 1 out]
          }
        }
        n181 = call-dynamic "Delacor_lib_QMH_Error Handler - Helper Loop.vi"("Error Debug"=w45, "error in"=w47, "Message Queue in"=w46) -> ()  [unwired: 7 in, 2 out]
      }
      n182 = Unregister For Events(event registration refnum=w28) -> ()  [unwired: 1 in, 1 out]
    }
    frame Error {
      n183 = call "Synchronize Caller Events.vi"("Module Admin"=w406) -> ("Module Admin out"=w405:refnum<class "Delacor_lib_QMH_Cloneable Module Admin.lvclass">)  [unwired: 9 in, 1 out]
      n184 = property on="Property Node" class="Mod Admin"(reference=w405) -> ("Accessors:Module ID"=w404:i32)  [unwired: 1 in, 2 out]
      n185 = call-dynamic "Delacor_lib_QMH_Release Message Queue.vi"("error in"=w412, "Message Queue"=w403) -> ("error out"=w411:errorcluster)  [unwired: 9 in]
      n186 = call "Module Name--constant.vi"("Module ID"=w404) -> ("Module Name"=w409:string)  [unwired: 10 in]
      n187 = Format Into String(format string="An error occurred during initialization. %s is no longer running.", w409) -> (resulting string=w407:string)  [unwired: 2 in, 1 out]
      n188 = call "Error Reported.vi"("Additional Information"=w407, "Error"=w411, "Module ID"=w404) -> ()  [unwired: 8 in, 1 out]
    }
  }
  n189 = Merge Errors(w21, w20) -> (w22:errorcluster)
  n190 = call "Close Module.vi"("error in"=w22, "Wait for stop?"=w9, "Module Admin in"=w3) -> ("error out"=w19:errorcluster, "External Launch"=w8:bool, "Module Admin out"=w10:refnum<class "Delacor_lib_QMH_Cloneable Module Admin.lvclass">)  [unwired: 6 in]
  n191 = call "clear-private-data.vi"("module-data"=w4) -> ()  [unwired: 10 in, 1 out]
  n192 = Unregister For Events(event registration refnum=w14, error in=w19) -> (error out=w18:errorcluster)
  "error out" <- w18
  n193 = local write "Module Admin"(w10) -> ()
  n194 = case "External Launch?" shown="True" w8 {
    tunnel: w18 -> [_ w413]
    frame False {
    }
    frame True {
      n195 = case shown="No Error" w413 {
        frame No Error {
          n196 = invoke class="VI" method="FP.Close"() -> ()  [unwired: 3 in, 3 out]
        }
        frame Error {
          n197 = invoke class="VI" method="FP.Open"("Activate"=TRUE ("Activate?")) -> ()  [unwired: 4 in, 5 out]
        }
      }
    }
  }
